vi "Module Identities.vi"(8 "error in (no error)":errorcluster, 11 "GUI Manager Module in":refnum<class "GUI Manager Module.lvclass">) -> (0 "error out":errorcluster, 2 "Identities":refnum<class "Identity.lvclass">[](array[class]), 3 "GUI Manager Module out":refnum<class "GUI Manager Module.lvclass">)   [LabVIEW 2020, in "VolatusGUI.lvlib" / "GUI Manager Module.lvclass"]
uses:
  GUI Manager Module.lvclass
  Volatus/Identity/Identity.lvclass
  Volatus/GUI Manager Identity/GUI Manager Identity.lvclass
  C:/dev/lv20CE/relink/lv-volatus/Volatus/Identity/Identity.lvclass
  GUI Manager Module.lvclass/GUI Manager Module.ctl
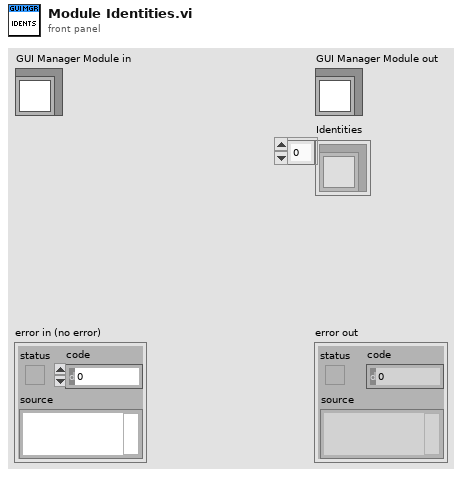
[diagram p1: front panel]
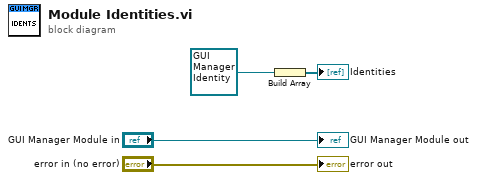
[diagram p0: block diagram]
diagram:
  n1 = Build Array(refnum<class "GUI Manager Identity.lvclass"> refnum ("VolatusGUI:GUI Manager Identity.lvclass")) -> (→"Identities":refnum<class "GUI Manager Identity.lvclass">[])
  "error out" <- "error in (no error)"
  "GUI Manager Module out" <- "GUI Manager Module in"
